vi "UE_Select_Setpoint.vi"(3 "default_target":dbl, 4 "override_target":dbl, 5 "override_selected":bool) -> (2 "selected_target":dbl)   [LabVIEW 2026]
doc: "INTENT: Select default or override target according to a validated mode flag. INPUTS: override_selected (bool), override_target (double), default_target (double). OUTPUTS: selected_target (double). DESIGN CONSTRAINT: REQUIREMENTS: SRS-F-019. No physical hardware side effects. Acceptance requires native LabVIEW compilation and behavioral testing."
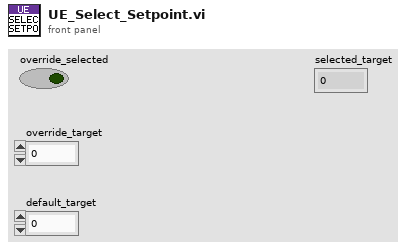
[diagram p1: front panel]
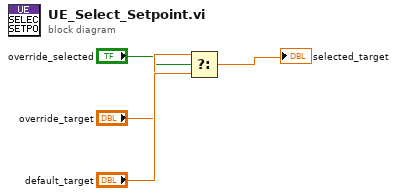
[diagram p0: block diagram]
diagram:
  n1 = Select(t="override_target", s="override_selected", f="default_target") -> (s? t:f=→"selected_target":dbl)
